vi "TCP Disconnect Client.vi"(8 "error in":errorcluster, 10 "connection ID":refnum<k5>, 11 "TCP Server":refnum<class "JKI TCP Server.lvclass">) -> (0 "error out":errorcluster)   [LabVIEW 2020, in "JKI TCP Server.lvclass"]
uses:
  JKI TCP Server.lvclass
  JKI TCP Server.lvclass/JKI TCP Server.ctl
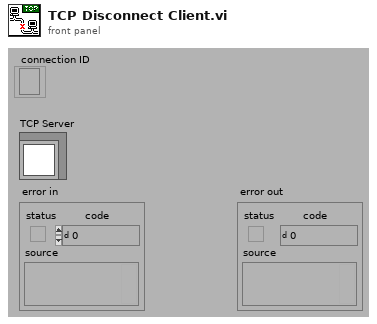
[diagram p1: front panel]
types:
  T1 = typedef "JKI TCP Server.lvclass/TCP Server Connection Info Cluster.ctl" = cluster{"connection ID":refnum<k5>, "Remote Address":string, "remote port":u16, "connection start time":u32}
  T2 = typedef "JKI TCP Server.lvclass/TCP Server Handler RefNum.ctl" = refnum<vi>
  T3 = cluster{"Connection Process VI Refnum":refnum<vi>, "TCP Handler VI RefNum":T2}
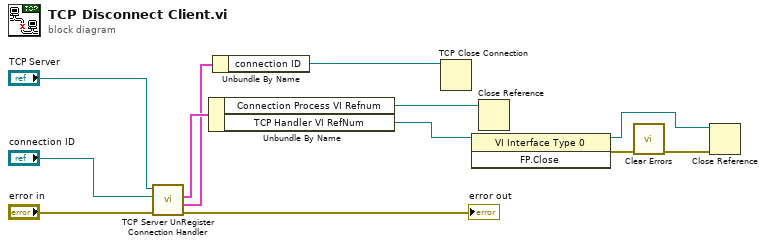
[diagram p0: block diagram]
diagram:
  n1 = call "TCP Server UnRegister Connection Handler.vi"("error in (no error)"="error in", "connection ID"="connection ID", "TCP Server RefNum"="TCP Server") -> ("error out"=→"error out":errorcluster, "Connection Info"=w10:T1, "VI References"=w11:T3)  [unwired: 6 out]
  n2 = Unbundle By Name(w11) -> ("Connection Process VI Refnum"=w5:refnum<vi>, "TCP Handler VI RefNum"=w4:T2)
  n3 = Unbundle By Name(w10) -> ("connection ID"=w12:refnum<k5>)
  n4 = TCP Close Connection(connection ID=w12) -> ()  [unwired: 1 in, 3 out]
  n5 = invoke class="VI Interface Type 0" method="FP.Close"(reference=w4) -> (reference out=w2:T2, error out=w3:errorcluster)  [unwired: 2 in, 1 out]
  n6 = Close Reference(reference=w5) -> ()  [unwired: 1 in, 1 out]
  n7 = call <vilib>:"Clear Errors.vi"("error in (no error)"=w3) -> ("error out"=w1:errorcluster)  [unwired: 1 in, 5 out]
  n8 = Close Reference(reference=w2, error in (no error)=w1) -> ()  [unwired: 1 out]
